vi "Probe lossy.vi"   [LabVIEW 2026]
doc: "Probe."
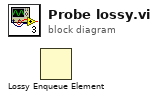
[diagram p0: block diagram]
diagram:
  n1 = Lossy Enqueue Element() -> ()  [unwired: 3 in, 4 out]
